vi "PLC_Link_Test.vi"() -> ()   [LabVIEW 2026]
doc: "Use this template to build a VI to use as a subVI."
panel:
  out "error out (code and source tell what failed)":errorcluster
  out "D230 X word, D231 Y word":u16[](array[numeric])
  out "4 PLC program running (D241 counts)":bool
  out "PLC Beat 2 (2 s later)":u16
  out "PLC Beat 1 (D241)":u16
  out "3 D241 read OK":bool
  out "2 PLC answers ENQ with ACK":bool
  out "1 Port opened":bool
  out "Resource used":string
  in  "Use Soft PLC (TCP 5551)":bool
  in  "COM Port (e.g. COM3)":string
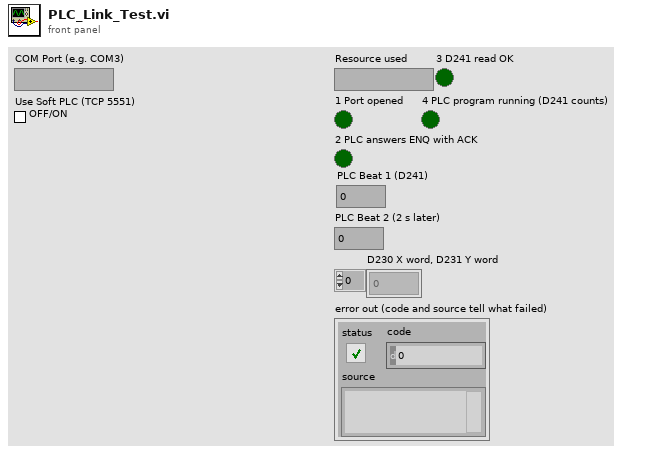
[diagram p1: front panel]
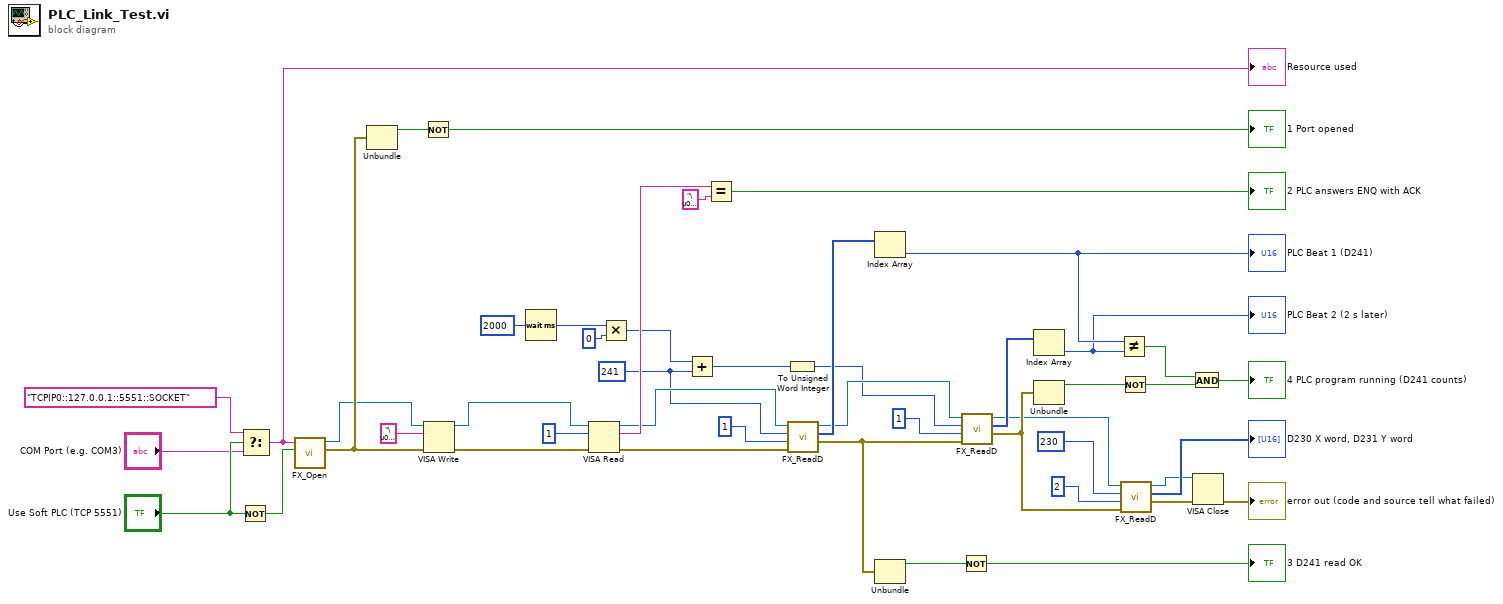
[diagram p0: block diagram]
diagram:
  w29 = 241
  n1 = Not(x="Use Soft PLC (TCP 5551)") -> (.not. x?=w43:bool)
  n2 = Select(t="TCPIP0::127.0.0.1::5551::SOCKET", s="Use Soft PLC (TCP 5551)", f="COM Port (e.g. COM3)") -> (s? t:f=w44:string)
  "Resource used" <- w44
  n3 = call "FX_Open.vi"("Serial (COM)?"=w43, "Resource"=w44) -> ("error out"=w42:errorcluster, "VISA out"=w39:refnum<visa-resource-name>)  [unwired: 8 in]
  n4 = Unbundle(w42) -> ("status"=w41:bool)  [unwired: 2 out]
  n5 = Not(x=w41) -> (.not. x?=→"1 Port opened":bool)
  n6 = VISA Write(VISA resource name=w39, write buffer="\u0005", error in (no error)=w42) -> (VISA resource name out=w37:refnum<visa-resource-name>, error out=w36:errorcluster)  [unwired: 1 out]
  n7 = Wait (ms)(milliseconds to wait=u32 2000) -> (millisecond timer value=w21:u32)
  n8 = VISA Read(VISA resource name=w37, byte count=u32 1, error in (no error)=w36) -> (VISA resource name out=w31:refnum<visa-resource-name>, read buffer=w34:string, error out=w30:errorcluster)  [unwired: 1 out]
  n9 = Multiply(x=w21, y=u32 0) -> (x*y=w19:u32)
  n10 = Add(x=w19, y=w29) -> (x+y=w18:u32)
  n11 = Equal?(x=w34, y="\u0006") -> (x = y?=→"2 PLC answers ENQ with ACK":bool)
  n12 = To Unsigned Word Integer(number=w18) -> (unsigned 16bit integer=w16:u16)
  n13 = call "FX_ReadD.vi"("error in (no error)"=w30, "Count"=u16 1, "D"=w29, "VISA in"=w31) -> ("error out"=w27:errorcluster, "Words"=w24:u16[], "VISA out"=w17:refnum<visa-resource-name>)  [unwired: 5 in]
  n14 = Index Array(array=w24) -> (element=w23:u16)  [unwired: 1 in]
  "PLC Beat 1 (D241)" <- w23
  n15 = Unbundle(w27) -> ("status"=w26:bool)  [unwired: 2 out]
  n16 = Not(x=w26) -> (.not. x?=→"3 D241 read OK":bool)
  n17 = call "FX_ReadD.vi"("error in (no error)"=w27, "Count"=u16 1, "D"=w16, "VISA in"=w17) -> ("error out"=w12:errorcluster, "Words"=w14:u16[], "VISA out"=w7:refnum<visa-resource-name>)  [unwired: 5 in]
  n18 = Index Array(array=w14) -> (element=w13:u16)  [unwired: 1 in]
  "PLC Beat 2 (2 s later)" <- w13
  n19 = Unbundle(w12) -> ("status"=w11:bool)  [unwired: 2 out]
  n20 = Not Equal?(x=w23, y=w13) -> (x != y?=w10:bool)
  n21 = Not(x=w11) -> (.not. x?=w9:bool)
  n22 = call "FX_ReadD.vi"("error in (no error)"=w12, "Count"=u16 2, "D"=230, "VISA in"=w7) -> ("error out"=w2:errorcluster, "Words"=→"D230 X word, D231 Y word":u16[], "VISA out"=w3:refnum<visa-resource-name>)  [unwired: 5 in]
  n23 = And(x=w10, y=w9) -> (x .and. y?=→"4 PLC program running (D241 counts)":bool)
  n24 = VISA Close(VISA resource name=w3, error in (no error)=w2) -> (error out=→"error out (code and source tell what failed)":errorcluster)
